vi "RemoteVI Check Track Modifiers.vi"() -> (4 "labels":string[](array[string]), 6 "expected":string[](array[string]), 8 "actual":string[](array[string]), 10 "failures":i32)   [LabVIEW 2020]
doc: "Test support, generated by tests/caraya/build.py from tests/vectors/translate.json (modifiers) - do not edit. Calls RemoteVI Track Modifiers.vi once per vector: the vector's input text goes through RemoteVI Parse Input.vi first, mods in is modsBefore, mods out is compared with modsAfter. Outputs, one element per vector: labels (the vector's name), expected (rendered from the vector), actual (the VI's result rendered the same way), and failures, the number of vectors whose expected and actual differ."
uses:
  source/RemoteVI.lvlib
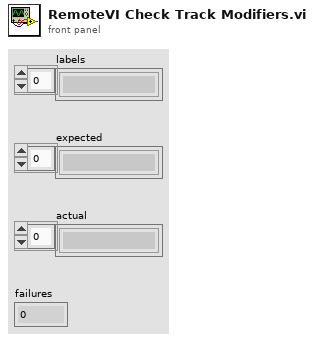
[diagram p1: front panel]
types:
  T1 = cluster{"name":string, "input":string, "modsBefore":u8, "expect":string}[]
  T2 = enum16{"invalid", "mouse", "key", "ack", "close", "splitter"}
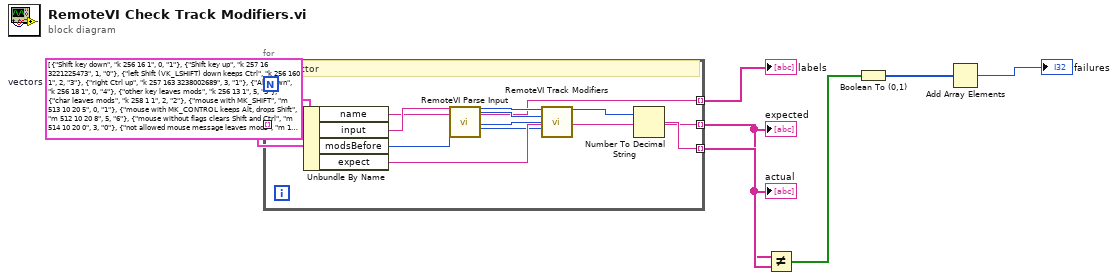
[diagram p0: block diagram]
diagram:
  w1 = T1 [{"name"="Shift key down", "input"="k 256 16 1", "modsBefore"=0, "expect"="1"}, {"name"="Shift key up", "input"="k 257 16 3221225473", "modsBefore"=1, "expect"="0"}, {"name"="left Shift (VK_LSHIFT) down keeps Ctrl", "input"="k 256 160 1", "modsBefore"=2, "expect"="3"}, {"name"="right Ctrl up", "input"="k 257 163 3238002689", "modsBefore"=3, "expect"="1"}, {"name"="Alt down", "input"="k 256 18 1", "modsBefore"=0, "expect"="4"}, {"name"="other key leaves mods", "input"="k 256 13 1", "modsBefore"=5, "expect"="5"}, {"name"="char leaves mods", "input"="k 258 1 1", "modsBefore"=2, "expect"="2"}, {"name"="mouse with MK_SHIFT", "input"="m 513 10 20 5", "modsBefore"=0, "expect"="1"}, {"name"="mouse with MK_CONTROL keeps Alt, drops Shift", "input"="m 512 10 20 8", "modsBefore"=5, "expect"="6"}, {"name"="mouse without flags clears Shift and Ctrl", "input"="m 514 10 20 0", "modsBefore"=3, "expect"="0"}, {"name"="not allowed mouse message leaves mods", "input"="m 16 1 1 0", "modsBefore"=3, "expect"="3"}, {"name"="ack leaves mods", "input"="a 5", "modsBefore"=1, "expect"="1"}]  # vectors
  n1 = for {
    tunnel: w1 -> [w8] mode=indexing
    tunnel: [w9] -> w2 mode=indexing
    tunnel: [w12] -> w3 mode=indexing
    tunnel: [w17] -> w4 mode=indexing
    # "One vector"
    n2 = Unbundle By Name(w8) -> ("name"=w9:string, "input"=w10:string, "modsBefore"=w11:u8, "expect"=w12:string)
    n3 = call "RemoteVI Parse Input.vi"("text"=w10) -> ("kind"=w13:T2, "msg"=w14:u32, "wParam"=w15:u64)  [unwired: 19 in, 5 out]
    n4 = call "RemoteVI Track Modifiers.vi"("kind"=w13, "msg"=w14, "wParam"=w15, "mods in"=w11) -> ("mods out"=w16:u8)  [unwired: 11 in]
    n5 = Number To Decimal String(number=w16) -> (decimal integer string=w17:string)  [unwired: 1 in]
  }
  "labels" <- w2
  "expected" <- w3
  "actual" <- w4
  n6 = Not Equal?(x=w3, y=w4) -> (x != y?=w5:bool[])
  n7 = Boolean To (0,1)(Boolean=w5) -> (0, 1=w6:i16[])
  n8 = Add Array Elements(numeric array=w6) -> (sum=→"failures":i16)
